vi "PSK Main.vi"() -> ()   [LabVIEW 2026]
panel:
  out "Recovered Binary Signal":dbl[](array[numeric])
  out "PSK Modulated Signal":dbl[](graph)
  out "Baseband Signal":dbl[](graph)
  in  "Phase for Binary 1":dbl
  in  "Amplitude(A)":dbl
  in  "Carrier Frequency(fc)":dbl
  in  "Bit Rate(Rb)":dbl
  in  "Sampling Frequency (Fs)":dbl
  in  "Binary Input":dbl[](array[numeric])
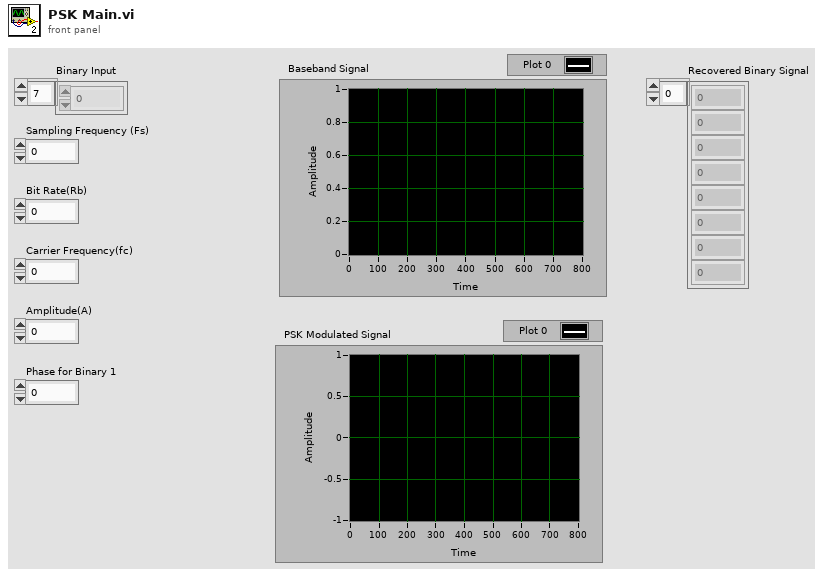
[diagram p1: front panel]
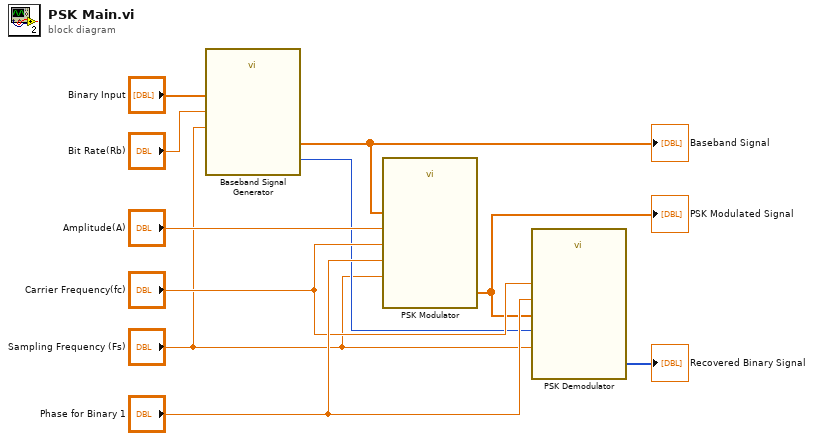
[diagram p0: block diagram]
diagram:
  n1 = call "Baseband Signal Generator.vi"("Bit Rate(Rb)"="Bit Rate(Rb)", "Sampling Frequency(Fs)"="Sampling Frequency (Fs)", "Binary Input"="Binary Input") -> ("Baseband Signal"=w1:dbl[], "Samples per bit"=w5:i32)
  "Baseband Signal" <- w1
  n2 = call "PSK Modulator.vi"("Baseband Signal"=w1, "Sampling Frequency(Fs)"="Sampling Frequency (Fs)", "Carrier Frequency (fc)"="Carrier Frequency(fc)", "Carrier Amplitude (A)"="Amplitude(A)", "Phase for Binary 1"="Phase for Binary 1") -> ("PSK Modulated Waveform"=w2:dbl[])
  "PSK Modulated Signal" <- w2
  n3 = call "PSK Demodulator.vi"("PSK Modulated Signal"=w2, "Sampling Frequency(Fs)"="Sampling Frequency (Fs)", "Carrier Frequency (fc)"="Carrier Frequency(fc)", "Samples per Bit"=w5, "Phase for Binary 1"="Phase for Binary 1") -> ("Recovered Binary Signal"=→"Recovered Binary Signal":i32[])
